vi "Serial Transmit Receive Simulation.vi"() -> ()   [LabVIEW 2013]
uses:
  <vilib>/rvi/DesktopExecutionNode/Execution/niFpgaDEN_Execute.vi
  <vilib>/rvi/DesktopExecutionNode/DesktopExecutionNode.xnode
  Source/I2S-TDM.lvlib
panel:
  out "sample out bits":bool[](array[boolean])
  in  "force stop":bool
  in  "ready for output":bool
  out "sample in":u32
  out "sample out":u32
  in  "start transfer":bool
  in  "pause":bool
  in  "24-bit data":bool[](array[boolean])=[TRUE, FALSE, FALSE, FALSE, FALSE, FALSE, FALSE, FALSE, FALSE, FALSE, FALSE, FALSE, FALSE, FALSE, FALSE, FALSE, FALSE, FALSE, FALSE, FALSE, FALSE, FALSE, FALSE, TRUE]
  in  "wait":u32=50
  out "Digital Waveform Graph":digitalwaveform(graph)
  in  "input valid":bool
  in  "transfer length":u8=32
  in  "stop":bool
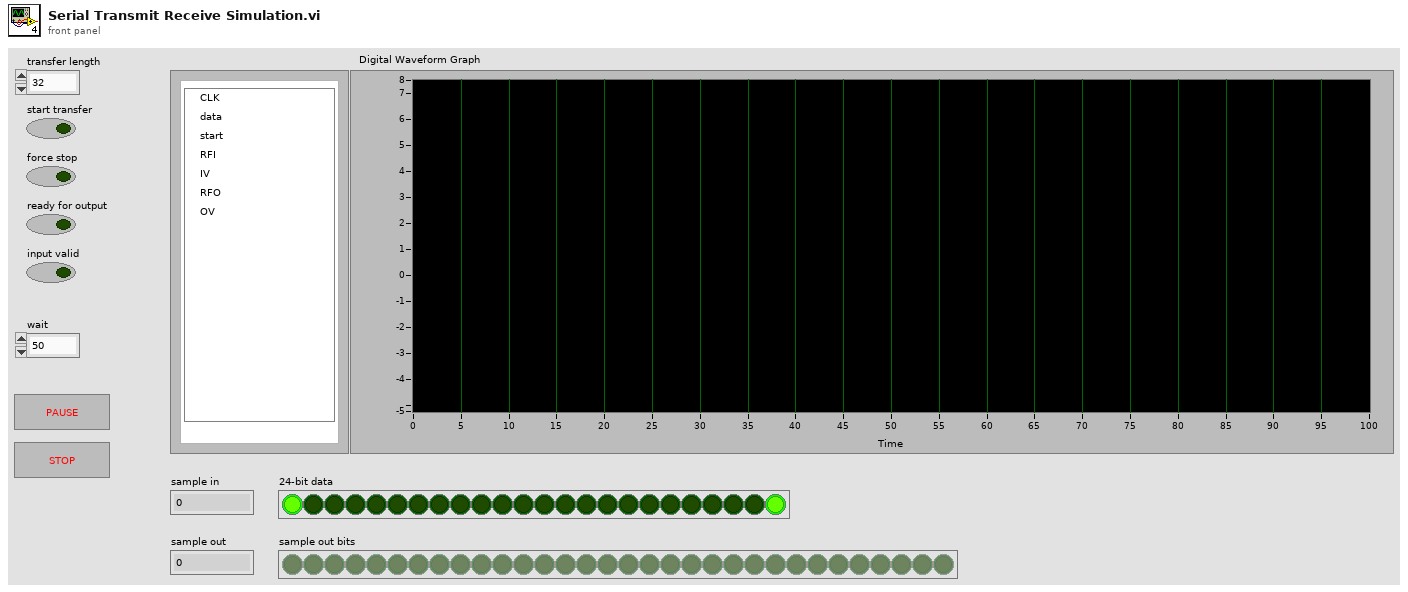
[diagram p1: front panel]
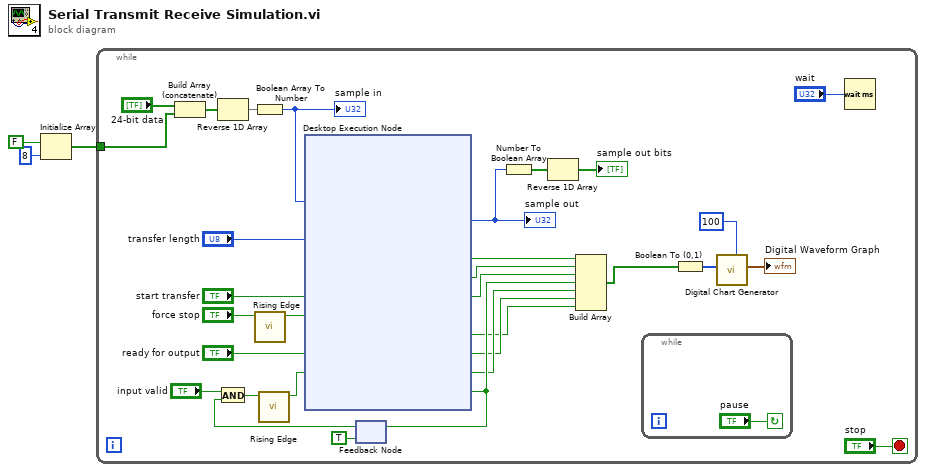
[diagram p0: block diagram]
diagram:
  n1 = Initialize Array(FALSE, 8 ("dimension size")) -> (w1:bool[])
  n2 = while {
    tunnel: w1 -> [w29]
    stop <- "stop" stop-if-true
    n3 = Build Array (concatenate)("24-bit data", w29) -> (w28:bool[])
    n4 = Reverse 1D Array(array=w28) -> (reversed array=w27:bool[])
    n5 = Boolean Array To Number(Boolean array=w27) -> (number=w23:u32)
    "sample in" <- w23
    n6 = call "Rising Edge.vi"("signal in"="force stop") -> ("rising edge?"=w4:bool)  [unwired: 10 in]
    n7 = feedback #1(TRUE ("ready for input")) -> (w19:bool)
    n8 = And(x="input valid", y=w19) -> (x .and. y?=w21:bool)
    n9 = call "Rising Edge.vi"("signal in"=w21) -> ("rising edge?"=w20:bool)  [unwired: 10 in]
    n10 = xnode "Desktop Execution Node"("sample in"=w23, "transfer length"="transfer length", "start transfer"="start transfer", "force stop"=w4, "ready for output"="ready for output", "input valid"=w20) -> ("sample out"=w10:u32, "clk"=w25:bool, "data"=w6:bool, "start transfer"=w7:bool, "output valid"=w13:bool, "ready for output"=w14:bool, "input valid"=w15:bool, "ready for input"=w16:bool)  [unwired: 1 in, 1 out]
    "sample out" <- w10
    n11 = feedback-in #1(w16) -> ()
    n12 = Number To Boolean Array(number=w10) -> (Boolean array=w9:bool[])
    n13 = Reverse 1D Array(array=w9) -> (reversed array=→"sample out bits":bool[])
    n14 = Build Array(w25, w6, w7, w16, w15, w14, w13) -> (w12:bool[])
    n15 = while {
      stop <- "pause" continue-if-true
    }
    n16 = Boolean To (0,1)(Boolean=w12) -> (0, 1=w11:i16[])
    n17 = call "Digital Chart Generator.vi"("History Size"=100, "Input"=w11) -> ("Digital Data"=→"Digital Waveform Graph":digitalwaveform)  [unwired: 9 in]
    n18 = Wait (ms)(milliseconds to wait="wait") -> ()  [unwired: 1 out]
  }
